vi "Create New Group.vi"(8 "error in (no error)":errorcluster, 11 "Selector in":refnum<class "Selector.lvclass">) -> (0 "error out":errorcluster, 1 "Group":string, 2 "Name":string, 3 "Selector out":refnum<class "Selector.lvclass">)   [LabVIEW 2019, in "Selector.lvclass"]
uses:
  Selector.lvclass
  Selector.lvclass/Selector.ctl
  cce5df9e-5964-4f11-9dff-719ececaf2a4.vi
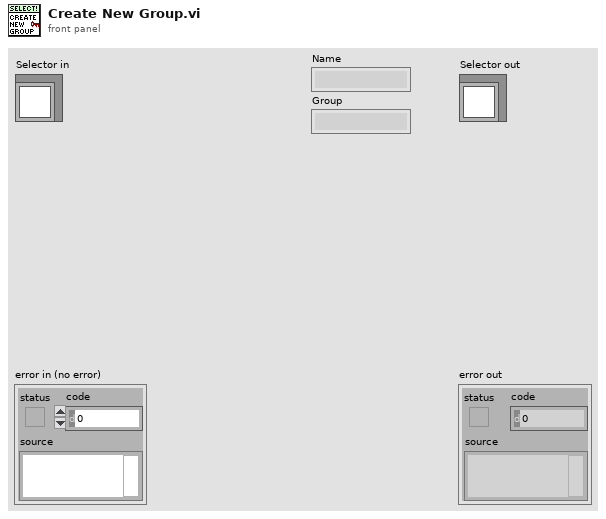
[diagram p1: front panel]
types:
  T1 = typedef "Selector.lvclass/Item.ctl" = cluster{"Name":string, "Group":string, "Enabled":bool}
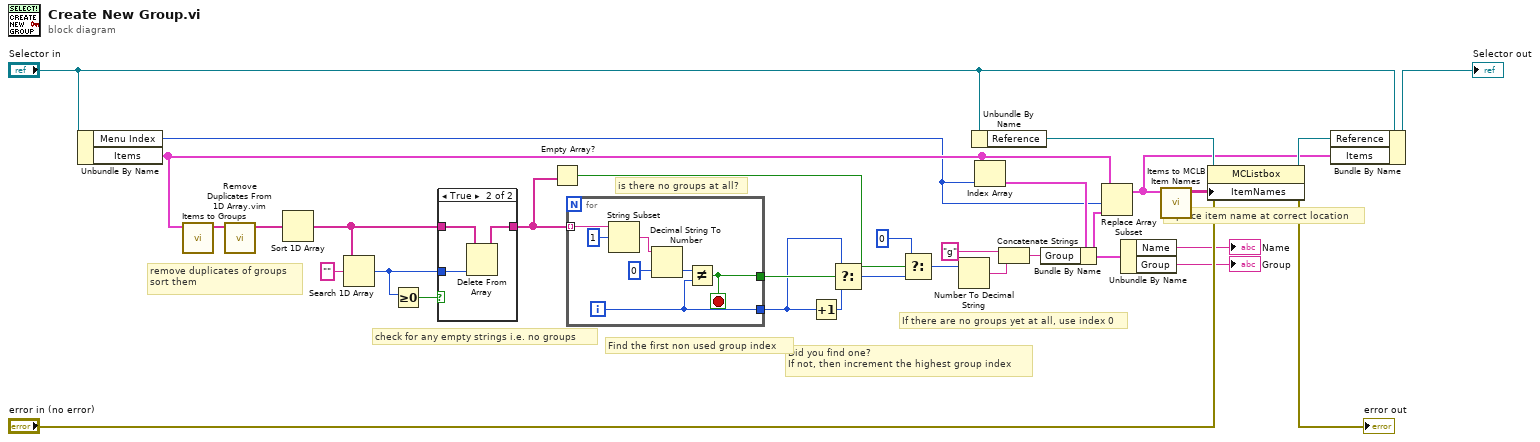
[diagram p0: block diagram]
diagram:
  # "replace item name at correct location"
  # "If there are no groups yet at all, use index 0"
  # "Did you find one?\nIf not, then increment the highest group index"
  # "Find the first non used group index"
  # "is there no groups at all?"
  # "check for any empty strings i.e. no groups"
  # "remove duplicates of groups\nsort them"
  n1 = Unbundle By Name("Selector in") -> ("Menu Index"=w4:i32, "Items"=w5:T1[])
  n2 = call "Items to Groups.vi"("Items"=w5) -> ("Groups"=w10:string[])  [unwired: 6 in]
  n3 = call "Remove Duplicates From 1D Array.vim"("array"=w10) -> ("array with duplicates removed"=w31:string[])  [unwired: 10 in]
  n4 = Sort 1D Array(array=w31) -> (sorted array=w21:string[])
  n5 = Search 1D Array(1D array=w21, element="") -> (index of element=w28:i32)  [unwired: 1 in]
  n6 = Greater Or Equal To 0?(x=w28) -> (x >= 0?=w29:bool)
  n7 = case shown="True" w29 {
    tunnel: w21 -> [w32 w35]
    tunnel: [w32 w34] -> w23
    tunnel: w28 -> [_ w33]
    frame False {
    }
    frame True {
      n8 = Delete From Array(array=w35, index=w33) -> (array with subset deleted=w34:string[])  [unwired: 1 in, 1 out]
    }
  }
  n9 = Empty Array?(array=w23) -> (empty?=w15:bool)
  n10 = for {
    tunnel: w23 -> [w37] mode=indexing
    tunnel: [w39] -> w27
    tunnel: [w36] -> w19
    i -> [w36]
    stop <- w39 stop-if-true
    n11 = String Subset(string=w37, offset (0)=1) -> (substring=w38:string)  [unwired: 1 in]
    n12 = Decimal String To Number(string=w38, default (0L)=0) -> (number=w40:i32)  [unwired: 1 in, 1 out]
    n13 = Not Equal?(x=w40, y=w36) -> (x != y?=w39:bool)
  }
  n14 = Increment(x=w19) -> (x+1=w20:i32)
  n15 = Select(t=w19, s=w27, f=w20) -> (s? t:f=w17:i32)
  n16 = Select(t=0, s=w15, f=w17) -> (s? t:f=w22:i32)
  n17 = Number To Decimal String(number=w22) -> (decimal integer string=w18:string)  [unwired: 1 in]
  n18 = Unbundle By Name("Selector in") -> ("Reference"=w25:refnum<vi>)
  n19 = Index Array(array=w5, index=w4) -> (element=w9:T1)
  n20 = Concatenate Strings("g" ("string"), w18) -> (w8:string)
  n21 = Bundle By Name(cluster=w9, "Group"=w8) -> (w3:T1)
  n22 = Replace Array Subset(array=w5, new element=w3, index=w4) -> (w6:T1[])
  n23 = Unbundle By Name(w3) -> ("Name"=→"Name":string, "Group"=→"Group":string)
  n24 = call "Items to MCLB Item Names.vi"("Items"=w6) -> ("Item Names"=w7:string[][])  [unwired: 6 in]
  n25 = property class="MCListbox"(reference=w25, error in="error in (no error)", "ItemNames"=w7) -> (reference out=w14:refnum<vi>, error out=→"error out":errorcluster)
  n26 = Bundle By Name(cluster="Selector in", "Reference"=w14, "Items"=w6) -> (→"Selector out":refnum<class "Selector.lvclass">)
